vi "Write Teller.vi"(10 "Teller":refnum<class "Teller.lvclass">, 11 "Stop Msg Input in":refnum<class "Stop Msg Input.lvclass">) -> (3 "Stop Msg Input out":refnum<class "Stop Msg Input.lvclass">)   [LabVIEW 2020, in "jettl.lvlib" / "Stop jettl Msg.lvlib" / "Stop Msg Input.lvlib" / "Stop Msg Input.lvclass"]
uses:
  Stop Msg Input.lvclass
  Teller/Teller.lvclass
  Stop Msg Input.lvclass/Stop Msg Input.ctl
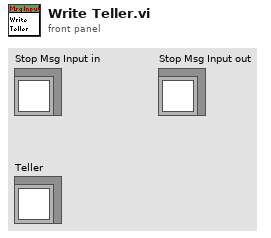
[diagram p1: front panel]
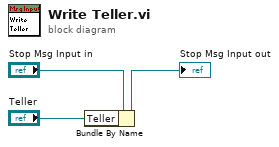
[diagram p0: block diagram]
diagram:
  n1 = Bundle By Name(cluster="Stop Msg Input in", "Teller"="Teller") -> (→"Stop Msg Input out":refnum<class "Stop Msg Input.lvclass">)
